vi "PicoScope5000aUnitInfo.vi"(3 "Mode":u16(ring) items=["Dialog On Error", "no dialog - CloseUnit and Stop", "no dialog - Continue", "no dialog - Stop"], 4 "handle in":i16, 5 "error in (no error)":errorcluster) -> (0 "Unit Info":T1, 1 "handle out":i16, 2 "error out":errorcluster)   [LabVIEW 2010]
uses:
  ps5000a.dll
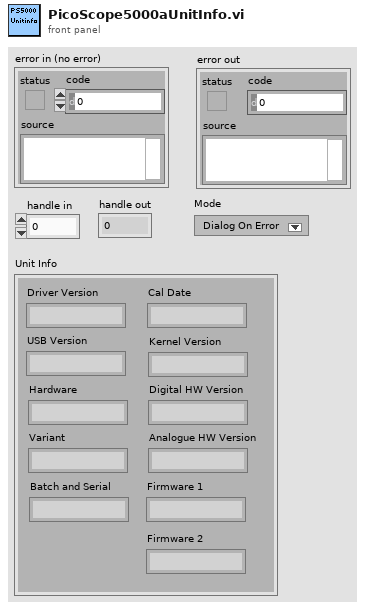
[diagram p1: front panel]
types:
  T1 = cluster{"Driver Version":string, "USB Version":string, "Hardware":string, "Variant":string, "Batch and Serial":string, "Cal Date":string, "Kernel Version":string, "Digital HW Version":string, "Analogue HW Version":string, "Firmware 1":string, "Firmware 2":string}
  T2 = cluster{"status":bool, "code":u32, "source":string}
  T3 = cluster{"[0]":string, "[1]":string, "[2]":string, "[3]":string, "[4]":string, "[5]":string, "[6]":string, "[7]":string, "[8]":string, "[9]":string, "[10]":string}
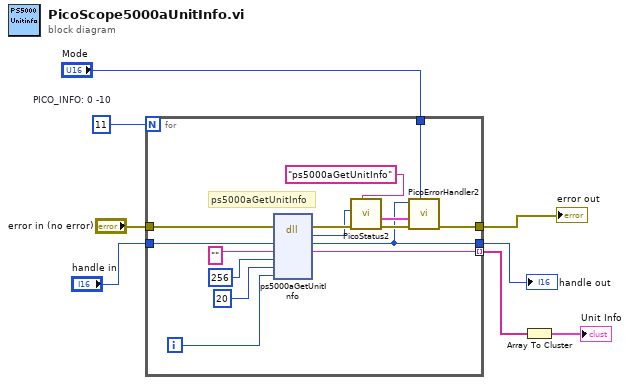
[diagram p0: block diagram]
diagram:
  w7 = 11  # PICO_INFO: 0 -10
  n1 = for {
    N: w7 -> [_]
    tunnel: "handle in" -> [w23]
    tunnel: [w20] -> w4 mode=indexing
    tunnel: "error in (no error)" -> [w17]
    tunnel: [w9] -> w5
    tunnel: [w13] -> w2
    tunnel: "Mode" -> [w10]
    i -> [w18]
    # "ps5000aGetUnitInfo"
    n2 = dll-call lib="ps5000a.dll" fn="ps5000aGetUnitInfo"(error in=w17, "handle"=w23, "unitInfo"="", "stringLength"=i16 256, "requiredSize"=i16 20 ("stringLength"), "pico_info"=w18) -> (error out=w12:errorcluster, "PICO_STATUS"=w11:u32, "handle"=w9:i16, "unitInfo"=w20:string)  [unwired: 5 in, 1 out]
    n3 = call "PicoStatus2.vi"("PICO source"="ps5000aGetUnitInfo" ("source"), "Error in"=w12, "PICO STATUS"=w11) -> ("error out"=w16:errorcluster, "PICO_STATUS out"=w15:T2)  [unwired: 5 in]
    n4 = call "PicoErrorHandler2.vi"("Mode"=w10, "error in (no error)"=w16, "PICO_STATUS in"=w15, "handle In"=w9) -> ("error out"=w13:errorcluster)  [unwired: 7 in]
  }
  "error out" <- w2
  "handle out" <- w5
  n5 = Array To Cluster(array=w4) -> (cluster=→"Unit Info":T3)
